vi "Validate Signed Representation Test Vectors.vi"() -> ()   [LabVIEW 2026, in "Utility.lvlib"]
doc: "Standalone test harness for signed-representation conversion. Replace placeholder actual result controls by wiring outputs from To Signed Representation.vim over each type test vector."
uses:
  Utility.lvlib
  Types/Signed Representation.ctl
  03fae9d8-b403-41ce-92e5-cc784c7a126a.vi
  78d6fb15-39c3-4b57-85ec-6913dbd0ca41.vi
  d45d5563-1e70-4b2e-af5d-47e39ffbbc8e.vi
  a2727b9d-4ec3-432e-bad0-44a54eeb1aee.vi
  03fae9d8-b403-41ce-92e5-cc784c7a126a.vi/fdd2035b-52a6-4314-93d5-e6d0012ea0d5.vi
  03fae9d8-b403-41ce-92e5-cc784c7a126a.vi/d7ddfa2c-0539-47bf-9b9d-3a470632982d.vi
  03fae9d8-b403-41ce-92e5-cc784c7a126a.vi/b8120071-ec88-4802-9c07-9d147ec9c255.vi
  03fae9d8-b403-41ce-92e5-cc784c7a126a.vi/96d3ddf9-193f-4353-8b9f-7b29ff2119cb.vi
  03fae9d8-b403-41ce-92e5-cc784c7a126a.vi/a2043324-c5a4-4327-a6d6-ab77c0f4b7eb.vi
  78d6fb15-39c3-4b57-85ec-6913dbd0ca41.vi/fdd2035b-52a6-4314-93d5-e6d0012ea0d5.vi
  78d6fb15-39c3-4b57-85ec-6913dbd0ca41.vi/d7ddfa2c-0539-47bf-9b9d-3a470632982d.vi
  78d6fb15-39c3-4b57-85ec-6913dbd0ca41.vi/b8120071-ec88-4802-9c07-9d147ec9c255.vi
  78d6fb15-39c3-4b57-85ec-6913dbd0ca41.vi/96d3ddf9-193f-4353-8b9f-7b29ff2119cb.vi
  78d6fb15-39c3-4b57-85ec-6913dbd0ca41.vi/a2043324-c5a4-4327-a6d6-ab77c0f4b7eb.vi
  d45d5563-1e70-4b2e-af5d-47e39ffbbc8e.vi/fdd2035b-52a6-4314-93d5-e6d0012ea0d5.vi
  d45d5563-1e70-4b2e-af5d-47e39ffbbc8e.vi/d7ddfa2c-0539-47bf-9b9d-3a470632982d.vi
  d45d5563-1e70-4b2e-af5d-47e39ffbbc8e.vi/b8120071-ec88-4802-9c07-9d147ec9c255.vi
  d45d5563-1e70-4b2e-af5d-47e39ffbbc8e.vi/96d3ddf9-193f-4353-8b9f-7b29ff2119cb.vi
  d45d5563-1e70-4b2e-af5d-47e39ffbbc8e.vi/a2043324-c5a4-4327-a6d6-ab77c0f4b7eb.vi
  a2727b9d-4ec3-432e-bad0-44a54eeb1aee.vi/fdd2035b-52a6-4314-93d5-e6d0012ea0d5.vi
  a2727b9d-4ec3-432e-bad0-44a54eeb1aee.vi/d7ddfa2c-0539-47bf-9b9d-3a470632982d.vi
  a2727b9d-4ec3-432e-bad0-44a54eeb1aee.vi/b8120071-ec88-4802-9c07-9d147ec9c255.vi
  a2727b9d-4ec3-432e-bad0-44a54eeb1aee.vi/96d3ddf9-193f-4353-8b9f-7b29ff2119cb.vi
  a2727b9d-4ec3-432e-bad0-44a54eeb1aee.vi/a2043324-c5a4-4327-a6d6-ab77c0f4b7eb.vi
  03fae9d8-b403-41ce-92e5-cc784c7a126a.vi/b8120071-ec88-4802-9c07-9d147ec9c255.vi/8ccb98a6-deb9-4b5a-be05-054c1c212d54.vi
  03fae9d8-b403-41ce-92e5-cc784c7a126a.vi/b8120071-ec88-4802-9c07-9d147ec9c255.vi/f171c548-4dcc-4c0c-949b-fc0df33543c2.vi
  03fae9d8-b403-41ce-92e5-cc784c7a126a.vi/b8120071-ec88-4802-9c07-9d147ec9c255.vi/d8adcdbd-60f3-48f3-8f6a-253ba0c2f91d.vi
  03fae9d8-b403-41ce-92e5-cc784c7a126a.vi/b8120071-ec88-4802-9c07-9d147ec9c255.vi/e61c01d5-f4be-4974-af39-63853a8697d8.vi
  03fae9d8-b403-41ce-92e5-cc784c7a126a.vi/96d3ddf9-193f-4353-8b9f-7b29ff2119cb.vi/8ccb98a6-deb9-4b5a-be05-054c1c212d54.vi
  03fae9d8-b403-41ce-92e5-cc784c7a126a.vi/96d3ddf9-193f-4353-8b9f-7b29ff2119cb.vi/f171c548-4dcc-4c0c-949b-fc0df33543c2.vi
  03fae9d8-b403-41ce-92e5-cc784c7a126a.vi/96d3ddf9-193f-4353-8b9f-7b29ff2119cb.vi/d8adcdbd-60f3-48f3-8f6a-253ba0c2f91d.vi
  03fae9d8-b403-41ce-92e5-cc784c7a126a.vi/96d3ddf9-193f-4353-8b9f-7b29ff2119cb.vi/e61c01d5-f4be-4974-af39-63853a8697d8.vi
  78d6fb15-39c3-4b57-85ec-6913dbd0ca41.vi/b8120071-ec88-4802-9c07-9d147ec9c255.vi/8ccb98a6-deb9-4b5a-be05-054c1c212d54.vi
  78d6fb15-39c3-4b57-85ec-6913dbd0ca41.vi/b8120071-ec88-4802-9c07-9d147ec9c255.vi/f171c548-4dcc-4c0c-949b-fc0df33543c2.vi
  78d6fb15-39c3-4b57-85ec-6913dbd0ca41.vi/b8120071-ec88-4802-9c07-9d147ec9c255.vi/d8adcdbd-60f3-48f3-8f6a-253ba0c2f91d.vi
  78d6fb15-39c3-4b57-85ec-6913dbd0ca41.vi/b8120071-ec88-4802-9c07-9d147ec9c255.vi/e61c01d5-f4be-4974-af39-63853a8697d8.vi
  78d6fb15-39c3-4b57-85ec-6913dbd0ca41.vi/96d3ddf9-193f-4353-8b9f-7b29ff2119cb.vi/8ccb98a6-deb9-4b5a-be05-054c1c212d54.vi
  78d6fb15-39c3-4b57-85ec-6913dbd0ca41.vi/96d3ddf9-193f-4353-8b9f-7b29ff2119cb.vi/f171c548-4dcc-4c0c-949b-fc0df33543c2.vi
  78d6fb15-39c3-4b57-85ec-6913dbd0ca41.vi/96d3ddf9-193f-4353-8b9f-7b29ff2119cb.vi/d8adcdbd-60f3-48f3-8f6a-253ba0c2f91d.vi
  78d6fb15-39c3-4b57-85ec-6913dbd0ca41.vi/96d3ddf9-193f-4353-8b9f-7b29ff2119cb.vi/e61c01d5-f4be-4974-af39-63853a8697d8.vi
  d45d5563-1e70-4b2e-af5d-47e39ffbbc8e.vi/b8120071-ec88-4802-9c07-9d147ec9c255.vi/8ccb98a6-deb9-4b5a-be05-054c1c212d54.vi
  d45d5563-1e70-4b2e-af5d-47e39ffbbc8e.vi/b8120071-ec88-4802-9c07-9d147ec9c255.vi/f171c548-4dcc-4c0c-949b-fc0df33543c2.vi
  d45d5563-1e70-4b2e-af5d-47e39ffbbc8e.vi/b8120071-ec88-4802-9c07-9d147ec9c255.vi/d8adcdbd-60f3-48f3-8f6a-253ba0c2f91d.vi
  d45d5563-1e70-4b2e-af5d-47e39ffbbc8e.vi/b8120071-ec88-4802-9c07-9d147ec9c255.vi/e61c01d5-f4be-4974-af39-63853a8697d8.vi
  d45d5563-1e70-4b2e-af5d-47e39ffbbc8e.vi/96d3ddf9-193f-4353-8b9f-7b29ff2119cb.vi/8ccb98a6-deb9-4b5a-be05-054c1c212d54.vi
  d45d5563-1e70-4b2e-af5d-47e39ffbbc8e.vi/96d3ddf9-193f-4353-8b9f-7b29ff2119cb.vi/f171c548-4dcc-4c0c-949b-fc0df33543c2.vi
  d45d5563-1e70-4b2e-af5d-47e39ffbbc8e.vi/96d3ddf9-193f-4353-8b9f-7b29ff2119cb.vi/d8adcdbd-60f3-48f3-8f6a-253ba0c2f91d.vi
  d45d5563-1e70-4b2e-af5d-47e39ffbbc8e.vi/96d3ddf9-193f-4353-8b9f-7b29ff2119cb.vi/e61c01d5-f4be-4974-af39-63853a8697d8.vi
  a2727b9d-4ec3-432e-bad0-44a54eeb1aee.vi/b8120071-ec88-4802-9c07-9d147ec9c255.vi/8ccb98a6-deb9-4b5a-be05-054c1c212d54.vi
  a2727b9d-4ec3-432e-bad0-44a54eeb1aee.vi/b8120071-ec88-4802-9c07-9d147ec9c255.vi/f171c548-4dcc-4c0c-949b-fc0df33543c2.vi
  a2727b9d-4ec3-432e-bad0-44a54eeb1aee.vi/b8120071-ec88-4802-9c07-9d147ec9c255.vi/d8adcdbd-60f3-48f3-8f6a-253ba0c2f91d.vi
  a2727b9d-4ec3-432e-bad0-44a54eeb1aee.vi/b8120071-ec88-4802-9c07-9d147ec9c255.vi/e61c01d5-f4be-4974-af39-63853a8697d8.vi
  a2727b9d-4ec3-432e-bad0-44a54eeb1aee.vi/96d3ddf9-193f-4353-8b9f-7b29ff2119cb.vi/8ccb98a6-deb9-4b5a-be05-054c1c212d54.vi
  a2727b9d-4ec3-432e-bad0-44a54eeb1aee.vi/96d3ddf9-193f-4353-8b9f-7b29ff2119cb.vi/f171c548-4dcc-4c0c-949b-fc0df33543c2.vi
  a2727b9d-4ec3-432e-bad0-44a54eeb1aee.vi/96d3ddf9-193f-4353-8b9f-7b29ff2119cb.vi/d8adcdbd-60f3-48f3-8f6a-253ba0c2f91d.vi
  a2727b9d-4ec3-432e-bad0-44a54eeb1aee.vi/96d3ddf9-193f-4353-8b9f-7b29ff2119cb.vi/e61c01d5-f4be-4974-af39-63853a8697d8.vi
panel:
  in  "i64 expected encoded":u64[](array[numeric])=[0, 1, 18446744073709551615, 9223372036854775808, 9223372036854775807, 1, 9223372036854775809, 18446744073709551615, 1, 18446744073709551614, 9223372036854775808]
  in  "i32 expected encoded":u32[](array[numeric])=[0, 1, 4294967295, 2147483648, 2147483647, 1, 2147483649, 4294967295, 1, 4294967294, 2147483648]
  in  "i16 expected encoded":u16[](array[numeric])=[0, 1, 65535, 32768, 32767, 1, 32769, 65535, 1, 65534, 32768]
  in  "expected valid":bool[](array[boolean])=[TRUE, TRUE, TRUE, TRUE, TRUE, TRUE, TRUE, FALSE, TRUE, TRUE, FALSE]
  in  "i8 expected encoded":u8[](array[numeric])=[0, 1, 255, 128, 127, 1, 129, 255, 1, 254, 128]
  out "all tests pass?":bool
  out "i64 pass?":bool
  in  "i64 test values":i64[](array[numeric])=[0, 1, -1, 0, -1, 1, -1, -9223372036854775808, 1, -1, -9223372036854775808]
  out "i32 pass?":bool
  in  "i32 test values":i32[](array[numeric])=[0, 1, -1, 0, -1, 1, -1, -2147483648, 1, -1, -2147483648]
  out "i16 pass?":bool
  in  "i16 test values":i16[](array[numeric])=[0, 1, -1, 0, -1, 1, -1, -32768, 1, -1, -32768]
  out "i8 pass?":bool
  in  "test encodings":T1[](array[typedef])=[enum."Two's Complement", enum."Two's Complement", enum."Two's Complement", enum."Offset Binary", enum."Offset Binary", enum."Sign-Magnitude", enum."Sign-Magnitude", enum."Sign-Magnitude", enum."Ones' Complement", enum."Ones' Complement", enum."Ones' Complement"]
  in  "i8 test values":i8[](array[numeric])=[0, 1, -1, 0, -1, 1, -1, -128, 1, -1, -128]
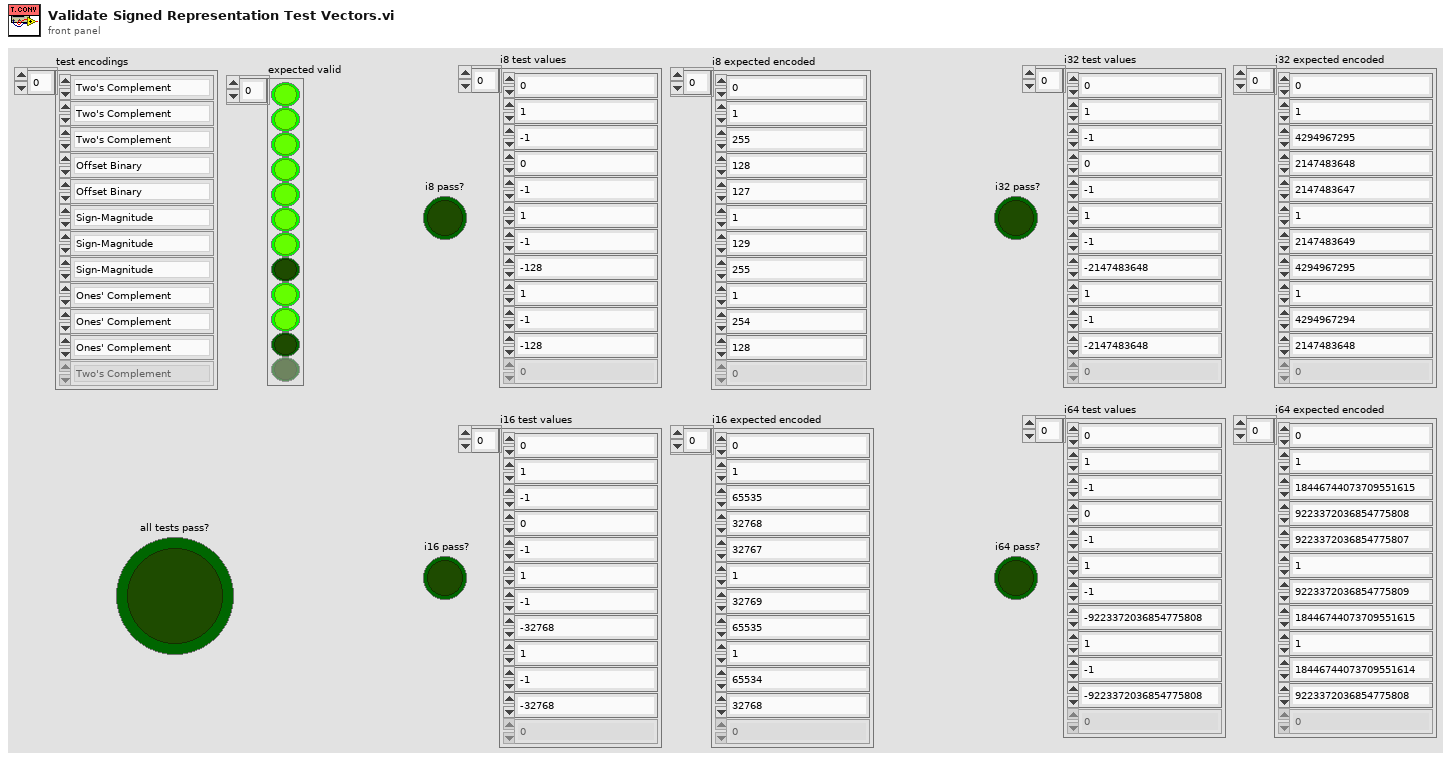
[diagram p1: front panel]
types:
  T1 = typedef "Utility.lvlib/Signed Representation.ctl" = enum16{"Two's Complement", "Offset Binary", "Sign-Magnitude", "Ones' Complement"}
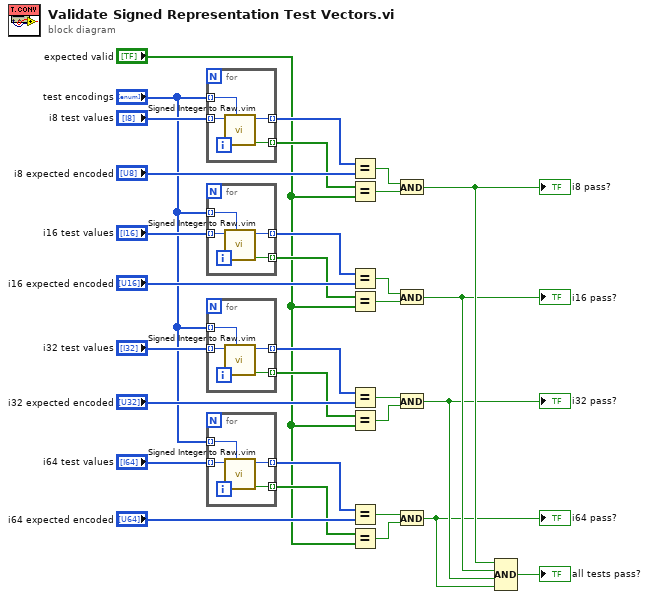
[diagram p0: block diagram]
diagram:
  n1 = for {
    tunnel: "test encodings" -> [w35] mode=indexing
    tunnel: "i8 test values" -> [w34] mode=indexing
    tunnel: [w33] -> w10 mode=indexing
    tunnel: [w32] -> w9 mode=indexing
    n2 = call "Signed Integer to Raw.vim"("Signed representation"=w35, "Value in"=w34) -> ("Valid?"=w32:bool, "Value (raw)"=w33:u8)  [unwired: 8 in]
  }
  n3 = for {
    tunnel: "test encodings" -> [w39] mode=indexing
    tunnel: "i16 test values" -> [w38] mode=indexing
    tunnel: [w37] -> w8 mode=indexing
    tunnel: [w36] -> w7 mode=indexing
    n4 = call "Signed Integer to Raw.vim"("Signed representation"=w39, "Value in"=w38) -> ("Valid?"=w36:bool, "Value (raw)"=w37:u16)  [unwired: 8 in]
  }
  n5 = for {
    tunnel: "test encodings" -> [w43] mode=indexing
    tunnel: "i32 test values" -> [w42] mode=indexing
    tunnel: [w41] -> w6 mode=indexing
    tunnel: [w40] -> w5 mode=indexing
    n6 = call "Signed Integer to Raw.vim"("Signed representation"=w43, "Value in"=w42) -> ("Valid?"=w40:bool, "Value (raw)"=w41:u32)  [unwired: 8 in]
  }
  n7 = for {
    tunnel: "test encodings" -> [w47] mode=indexing
    tunnel: "i64 test values" -> [w46] mode=indexing
    tunnel: [w45] -> w4 mode=indexing
    tunnel: [w44] -> w3 mode=indexing
    n8 = call "Signed Integer to Raw.vim"("Signed representation"=w47, "Value in"=w46) -> ("Valid?"=w44:bool, "Value (raw)"=w45:u64)  [unwired: 8 in]
  }
  n9 = Equal?(x=w10, y="i8 expected encoded") -> (x = y?=w30:bool)
  n10 = Equal?(x=w9, y="expected valid") -> (x = y?=w29:bool)
  n11 = Equal?(x=w8, y="i16 expected encoded") -> (x = y?=w27:bool)
  n12 = Equal?(x=w7, y="expected valid") -> (x = y?=w26:bool)
  n13 = Equal?(x=w6, y="i32 expected encoded") -> (x = y?=w24:bool)
  n14 = Equal?(x=w5, y="expected valid") -> (x = y?=w23:bool)
  n15 = Equal?(x=w4, y="i64 expected encoded") -> (x = y?=w21:bool)
  n16 = Equal?(x=w3, y="expected valid") -> (x = y?=w20:bool)
  n17 = And(x=w30, y=w29) -> (x .and. y?=w18:bool)
  "i8 pass?" <- w18
  n18 = And(x=w27, y=w26) -> (x .and. y?=w17:bool)
  "i16 pass?" <- w17
  n19 = And(x=w24, y=w23) -> (x .and. y?=w16:bool)
  "i32 pass?" <- w16
  n20 = And(x=w21, y=w20) -> (x .and. y?=w15:bool)
  "i64 pass?" <- w15
  n21 = Compound Arithmetic op=AND(w18, w17, w16, w15) -> (→"all tests pass?":bool)
